vi "VIH ProjFile - Group Rule - Write.vi"(6 "MasterRule (F)":bool, 8 "error in":errorcluster, 9 "Group Rule":T1, 10 "Project Folder":path, 11 "XML Parent Item":refnum<k20>) -> (0 "error out":errorcluster, 3 "dup XML Parent Item":refnum<k20>)   [LabVIEW 2014]
doc: "::: VI Helpeks :::\nCopyright (c) 2000-2026 Konstantin Shifershteyn. All rights reserved."
uses:
  _VIH HelpGen.llb/VIH HelpGen Typedef - Cluster - Group Rule.ctl
  _VIH HelpGen.llb/VIH HelpGen Typedef - Enum - Default,Enable,Disable.ctl
  _VIH HelpGen.llb/VIH HelpGen Typedef - Cluster - Group Rule - Source Paths.ctl
  _VIH HelpGen.llb/VIH HelpGen Typedef - Cluster - Group Rule - Target Paths.ctl
  _VIH HelpGen.llb/VIH HelpGen Typedef - Enum - Description Mode.ctl
  _VIH HelpGen.llb/VIH HelpGen Typedef - Cluster - Control Rule.ctl
  _VIH HelpGen.llb/VIH HelpGen Typedef - Cluster - Enum Value Info.ctl
  _VIH HelpGen.llb/VIH HelpGen Typedef - Cluster - Group Rule - Flags.ctl
  <vilib>/xml/Close Reference(Node).vi
  <resource>/objmgr/DOMUserDefRef.rc
  <vilib>/xml/NI_XML.lvlib
panel:
  in  "Group Rule (data)":T1
  # "VI Helpeks\nCopyright (c) 2012-2026 Konstantin Shifershteyn"
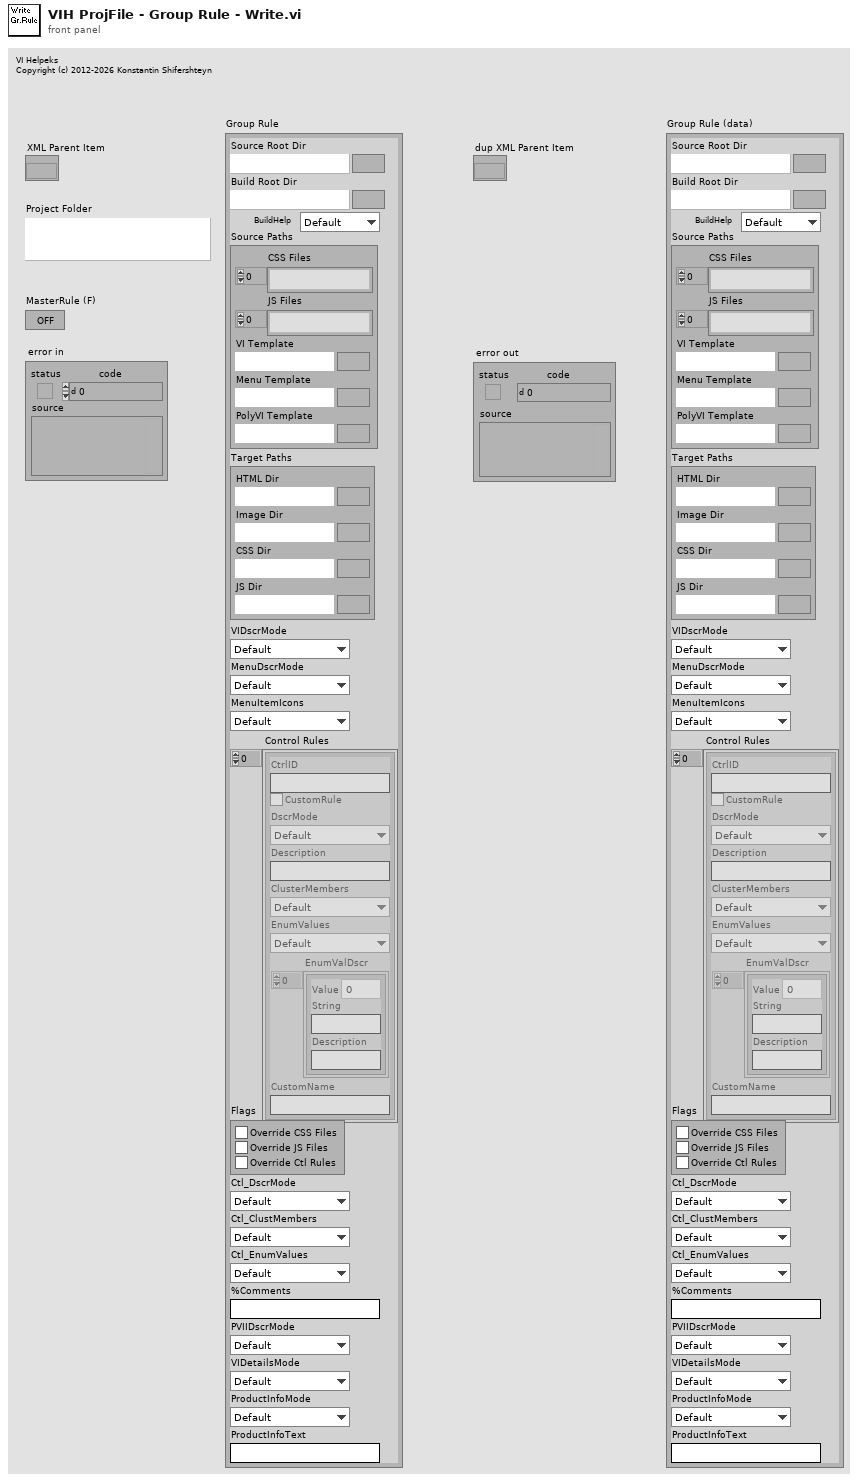
[diagram p1: front panel]
types:
  T1 = typedef "VIH HelpGen Typedef - Cluster - Group Rule.ctl" = cluster{"Source Root Dir":path, "Build Root Dir":path, "BuildHelp":T2, "Source Paths":T3, "Target Paths":T4, "VIDscrMode":T5, "MenuDscrMode":T5, "MenuItemIcons":T2, "Control Rules":T6[], "Flags":T8, "Ctl_DscrMode":T5, "Ctl_ClustMembers":T2, "Ctl_EnumValues":T2, "%Comments":string, "PVIIDscrMode":T5, "VIDetailsMode":T5, "ProductInfoMode":T2, "ProductInfoText":string}
  T2 = typedef "VIH HelpGen Typedef - Enum - Default,Enable,Disable.ctl" = enum16{"Default", "Enable", "Disable"}
  T3 = typedef "VIH HelpGen Typedef - Cluster - Group Rule - Source Paths.ctl" = cluster{"CSS Files":path[], "JS Files":path[], "VI Template":path, "Menu Template":path, "PolyVI Template":path}
  T4 = typedef "VIH HelpGen Typedef - Cluster - Group Rule - Target Paths.ctl" = cluster{"HTML Dir":path, "Image Dir":path, "CSS Dir":path, "JS Dir":path}
  T5 = typedef "VIH HelpGen Typedef - Enum - Description Mode.ctl" = enum16{"Default", "Description", "Description1", "Description2", "Custom", "None"}
  T6 = typedef "VIH HelpGen Typedef - Cluster - Control Rule.ctl" = cluster{"CtrlID":string, "CustomRule":bool, "DscrMode":T5, "Description":string, "ClusterMembers":T2, "EnumValues":T2, "EnumValDscr":T7[], "CustomName":string}
  T7 = typedef "VIH HelpGen Typedef - Cluster - Enum Value Info.ctl" = cluster{"Value":ext, "String":string, "Description":string}
  T8 = typedef "VIH HelpGen Typedef - Cluster - Group Rule - Flags.ctl" = cluster{"Override CSS Files":bool, "Override JS Files":bool, "Override Ctl Rules":bool}
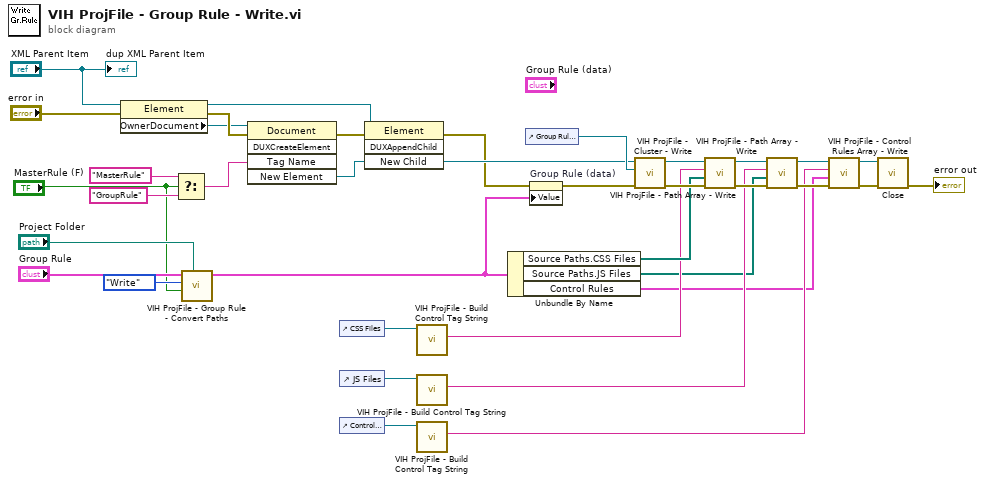
[diagram p0: block diagram]
diagram:
  n1 = property class="Element"(reference="XML Parent Item", error in="error in") -> (reference out=w11:refnum<k20>, error out=w13:errorcluster, "OwnerDocument"=w7:refnum<k20>)
  n2 = Select(t="MasterRule" ("Tag Name"), s="MasterRule (F)", f="GroupRule") -> (s? t:f=w8:string)
  n3 = call "VIH ProjFile - Group Rule - Convert Paths.vi"("Root Dir"="Project Folder", "Master Rule (F)"="MasterRule (F)", "Operation"=enum16{"Read", "Write"}."Write", "Group Rule"="Group Rule") -> ("Group Rule out"=w4:T1)  [unwired: 7 in]
  n4 = invoke class="Document" method="DUXCreateElement"(reference=w7, error in=w13, "Tag Name"=w8) -> (error out=w15:errorcluster, "New Element"=w35:refnum<k20>)  [unwired: 2 in, 3 out]
  n5 = control-ref of="CSS Files"() -> (w17:refnum<vi>)
  n6 = control-ref of="JS Files"() -> (w16:refnum<vi>)
  n7 = control-ref of="Control Rules"() -> (w6:refnum<vi>)
  n8 = invoke class="Element" method="DUXAppendChild"(reference=w11, error in=w15, "New Child"=w35) -> (error out=w33:errorcluster)  [unwired: 1 in, 3 out]
  n9 = call "VIH ProjFile - Build Control Tag String.vi"("Ctl Refnum"=w17) -> ("Control Tag"=w28:string)  [unwired: 6 in, 4 out]
  n10 = call "VIH ProjFile - Build Control Tag String.vi"("Ctl Refnum"=w16) -> ("Control Tag"=w25:string)  [unwired: 6 in, 4 out]
  n11 = call "VIH ProjFile - Build Control Tag String.vi"("Ctl Refnum"=w6) -> ("Control Tag"=w19:string)  [unwired: 6 in, 4 out]
  n12 = Unbundle By Name(w4) -> ("Source Paths.CSS Files"=w29:path[], "Source Paths.JS Files"=w24:path[], "Control Rules"=w18:T6[])
  n13 = control-ref of="Group Rule (data)"() -> (w36:refnum<vi>)
  n14 = property on="Group Rule (data)" class="Clust (strict)"(error in=w33, "Value"=w4) -> (error out=w34:errorcluster)  [unwired: 1 in, 1 out]
  n15 = call "VIH ProjFile - Cluster - Write.vi"("error in"=w34, "Ctl Refnum"=w36, "XML Parent Item"=w35) -> ("error out"=w30:errorcluster, "dup XML Parent Item"=w31:refnum<k20>)  [unwired: 7 in]
  n16 = call "VIH ProjFile - Path Array - Write.vi"("error in"=w30, "Paths"=w29, "Property Name"=w28, "XML Parent Item"=w31) -> ("error out"=w26:errorcluster, "dup XML Parent Item"=w27:refnum<k20>)  [unwired: 6 in]
  n17 = call "VIH ProjFile - Path Array - Write.vi"("error in"=w26, "Paths"=w24, "Property Name"=w25, "XML Parent Item"=w27) -> ("error out"=w22:errorcluster, "dup XML Parent Item"=w23:refnum<k20>)  [unwired: 6 in]
  n18 = call "VIH ProjFile - Control Rules Array - Write.vi"("error in"=w22, "Control Rules"=w18, "Property Name"=w19, "XML Parent Item"=w23) -> ("error out"=w21:errorcluster, "dup XML Parent Item"=w20:refnum<k20>)  [unwired: 6 in]
  n19 = call-poly <vilib>:"Close.vi"("error in (no error)"=w21, "node"=w20) -> ("error out"=→"error out":errorcluster)  [unwired: 7 in]
  "dup XML Parent Item" <- "XML Parent Item"
